vi "CE ExNav - Display Formatted Text in String Control.vi"(8 "error in":errorcluster, 10 "Formatted text":string, 11 "Str Refnum":refnum<vi>) -> (0 "error out":errorcluster, 3 "dup Str Refnum":refnum<vi>)   [LabVIEW 2021]
doc: "::: CalcExpress Toolkit :::\nCopyright (c) 2000-2026 Konstantin Shifershteyn. All rights reserved."
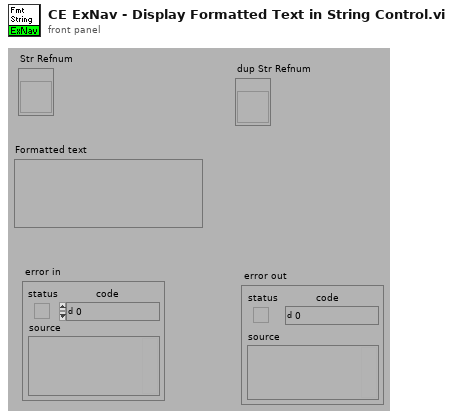
[diagram p1: front panel]
types:
  T1 = cluster{"Selection Start":u32, "Selection End":i32}
  T2 = cluster{"offset past replacement":i32, "offset past replacement":i32}
  T3 = cluster{"offset past replacement":i32, "offset past replacement":i32}[]
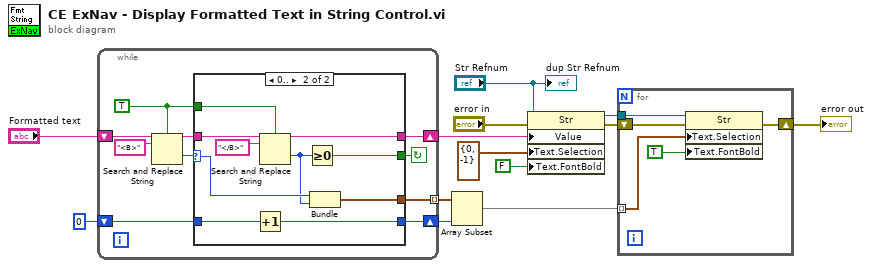
[diagram p0: block diagram]
diagram:
  n1 = while {
    shift-right: [w20] -> w6
    shift-left: "Formatted text" -> [w23]
    tunnel: [w17] -> w12 mode=indexing
    shift-right: [w15] -> w11
    shift-left: 0 -> [w14]
    stop <- w16 continue-if-true
    w18 = TRUE
    n2 = Search and Replace String(case sensitive?=w18, input string=w23, search string="<B>" ("search string/char (-)")) -> (result string=w19:string, offset past replacement=w21:i32)  [unwired: 5 in, 2 out]
    n3 = case shown="0.." w21 {
      selector: w21 -> [_ w31]
      tunnel: [w25 w27] -> w20
      tunnel: w19 -> [w25 w35]
      tunnel: w18 -> [_ w33]
      tunnel: [_ w32] -> w17
      tunnel: [_ w28] -> w16
      tunnel: [w24 w29] -> w15
      tunnel: w14 -> [w24 w30]
      frame ..-1 {
      }
      frame 0.. {
        n4 = Increment(x=w30) -> (x+1=w29:i32)
        n5 = Search and Replace String(case sensitive?=w33, input string=w35, search string="</B>" ("search string/char (-)")) -> (result string=w27:string, offset past replacement=w26:i32)  [unwired: 5 in, 2 out]
        n6 = Greater Or Equal To 0?(x=w26) -> (x >= 0?=w28:bool)
        n7 = Bundle("offset past replacement"=w31, "offset past replacement"=w26) -> (w32:T2)  [unwired: 1 in]
      }
    }
  }
  n8 = Array Subset(array=w12, length=w11) -> (w8:T3)  [unwired: 1 in]
  n9 = property class="Str"(reference="Str Refnum", error in="error in", "Value"=w6, "Text.Selection"=T1 {"Selection Start"=0, "Selection End"=-1}, "Text.FontBold"=FALSE) -> (reference out=w9:refnum<vi>, error out=w4:errorcluster)
  n10 = for {
    tunnel: w9 -> [w40]
    tunnel: w8 -> [w39] mode=indexing
    shift-right: [w36] -> w3
    shift-left: w4 -> [w37]
    n11 = property class="Str"(reference=w40, error in=w37, "Text.Selection"=w39, "Text.FontBold"=TRUE) -> (error out=w36:errorcluster)  [unwired: 1 out]
  }
  "error out" <- w3
  "dup Str Refnum" <- "Str Refnum"
